vi "test Add and Get Timing Channels.vi"(8 "error in":errorcluster, 11 "TestCase in":refnum<class "Scripting.lvclass">) -> (0 "error out":errorcluster)   [LabVIEW 2020, in "Scripting.lvclass"]
uses:
  Scripting.lvclass
  <vilib>/addons/_JKI Toolkits/VI Tester/TestCase.llb/TestCase.lvclass
  Scripting/Ballard/Ballard ARINC 429 Scripting.lvlib
  <vilib>/NI VeriStand/Custom Device API/Custom Device Item Ref.ctl
  <vilib>/NI VeriStand/Custom Device API/Custom Device API.lvlib
  C:/Program Files (x86)/National Instruments/LabVIEW 2020/vi.lib/addons/_JKI Toolkits/VI Tester/TestCase.llb/TestCase.lvclass
  C:/Users/nitest/Desktop/Git 2020/niveristand-ballard-arinc429-custom-device/Source/Custom Device Support/Tests/Unit/Scripting/Scripting.lvclass
panel:
  out "TestCase out":refnum<class "Scripting.lvclass">
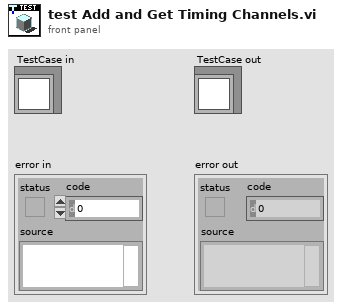
[diagram p1: front panel]
types:
  T1 = typedef "Custom Device API.lvlib/Custom Device Item Ref.ctl" = u64
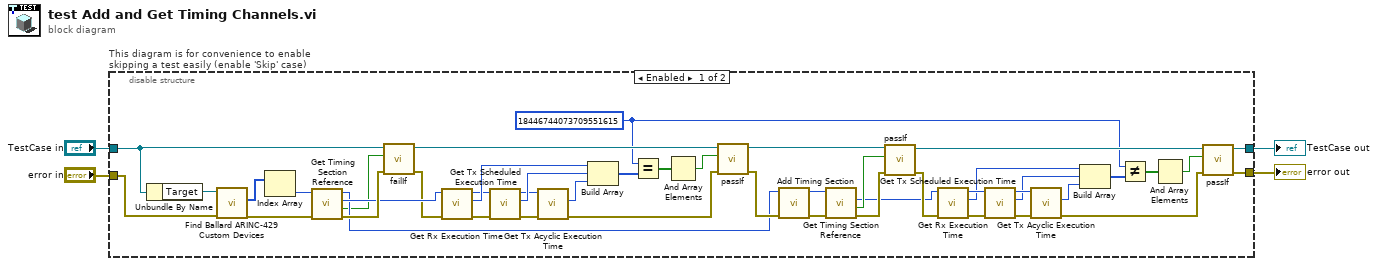
[diagram p0: block diagram]
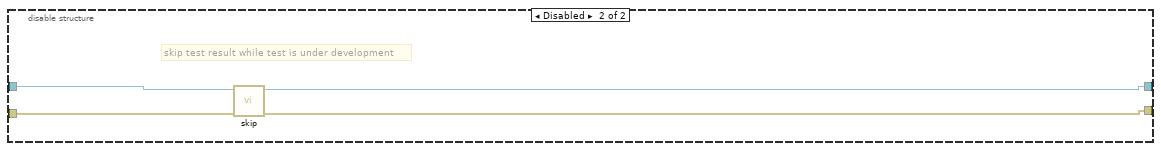
[diagram p2: hidden frame]
diagram:
  n1 = disable-structure "This diagram is for convenience to enable skipping a test easily (enable 'Skip' case)" shown="Enabled" {
    disable-tunnel: "TestCase in" -> [w50 w54]
    disable-tunnel: [w19 w52] -> w1
    disable-tunnel: [w20 w53] -> w3
    disable-tunnel: "error in" -> [w48 w51]
    frame Enabled {
      w5 = T1 18446744073709551615 ("tx acyclic execution time ref")
      n2 = Unbundle By Name(w50) -> ("Target"=w49:refnum<k24>)
      n3 = call "Find Ballard ARINC-429 Custom Devices.vi"("error in"=w48, "target in"=w49) -> ("error out"=w45:errorcluster, "Ballard ARINC 429 custom devices"=w47:u64[])  [unwired: 7 in, 1 out]
      n4 = Index Array(array=w47) -> (element=w46:u64)  [unwired: 1 in]
      n5 = call "Get Timing Section Reference.vi"("error in"=w45, "Ballard ARINC 429 ref"=w46) -> ("error out"=w44:errorcluster, "found"=w18:bool, "timing section ref"=w39:T1, "Ballard ARINC 429 ref out"=w32:T1)  [unwired: 6 in]
      n6 = call-dynamic "failIf.vi"("error in (no error)"=w44, "fail"=w18, "TestCase in"=w50) -> ("error out"=w14:errorcluster, "TestCase out"=w38:refnum<class "Scripting.lvclass">)  [unwired: 7 in]
      n7 = call "Get Rx Execution Time.vi"("error in"=w14, "timing section in"=w39) -> ("error out"=w41:errorcluster, "rx execution time ref"=w36:T1, "timing section out"=w25:T1)  [unwired: 7 in]
      n8 = call "Get Tx Scheduled Execution Time.vi"("error in"=w41, "timing section in"=w25) -> ("error out"=w40:errorcluster, "tx scheduled execution time ref"=w35:T1, "timing section out"=w24:T1)  [unwired: 7 in]
      n9 = call "Get Tx Acyclic Execution Time.vi"("error in"=w40, "timing section in"=w24) -> ("error out"=w37:errorcluster, "tx acyclic execution time ref"=w34:T1)  [unwired: 7 in, 1 out]
      n10 = Build Array(w36, w35, w34) -> (w11:T1[])
      n11 = Equal?(x=w5, y=w11) -> (x = y?=w10:bool[])
      n12 = And Array Elements(Boolean array=w10) -> (logical AND=w9:bool)
      n13 = call-dynamic "passIf.vi"("error in (no error)"=w37, "pass"=w9, "TestCase in"=w38) -> ("error out"=w33:errorcluster, "TestCase out"=w31:refnum<class "Scripting.lvclass">)  [unwired: 7 in]
      n14 = call "Add Timing Section.vi"("error in"=w33, "custom device ref"=w32) -> ("error out"=w43:errorcluster, "custom device ref out"=w42:T1)  [unwired: 7 in, 1 out]
      n15 = call "Get Timing Section Reference.vi"("error in"=w43, "Ballard ARINC 429 ref"=w42) -> ("error out"=w29:errorcluster, "found"=w17:bool, "timing section ref"=w12:T1)  [unwired: 6 in, 1 out]
      n16 = call-dynamic "passIf.vi"("error in (no error)"=w29, "pass"=w17, "TestCase in"=w31) -> ("error out"=w13:errorcluster, "TestCase out"=w16:refnum<class "Scripting.lvclass">)  [unwired: 7 in]
      n17 = call "Get Rx Execution Time.vi"("error in"=w13, "timing section in"=w12) -> ("error out"=w30:errorcluster, "rx execution time ref"=w23:T1, "timing section out"=w27:T1)  [unwired: 7 in]
      n18 = call "Get Tx Scheduled Execution Time.vi"("error in"=w30, "timing section in"=w27) -> ("error out"=w28:errorcluster, "tx scheduled execution time ref"=w22:T1, "timing section out"=w26:T1)  [unwired: 7 in]
      n19 = call "Get Tx Acyclic Execution Time.vi"("error in"=w28, "timing section in"=w26) -> ("error out"=w15:errorcluster, "tx acyclic execution time ref"=w21:T1)  [unwired: 7 in, 1 out]
      n20 = Build Array(w23, w22, w21) -> (w6:T1[])
      n21 = Not Equal?(x=w5, y=w6) -> (x != y?=w8:bool[])
      n22 = And Array Elements(Boolean array=w8) -> (logical AND=w7:bool)
      n23 = call-dynamic "passIf.vi"("error in (no error)"=w15, "pass"=w7, "TestCase in"=w16) -> ("error out"=w20:errorcluster, "TestCase out"=w19:refnum<class "Scripting.lvclass">)  [unwired: 7 in]
    }
    frame Disabled {
      # "skip test result while test is under development"
      n24 = call <vilib>:"skip.vi"("error in (no error)"=w51, "TestCase in"=w54) -> ("error out"=w53:errorcluster, "TestCase out"=w52:refnum<class "Scripting.lvclass">)  [unwired: 8 in]
    }
  }
  "error out" <- w3
  "TestCase out" <- w1
